vi "pallindrome.vi"() -> ()   [LabVIEW 2018]
panel:
  out "Numeric":dbl
  out "PALLINDROME OR NOT":string
  out "Boolean":bool
  in  "String":string
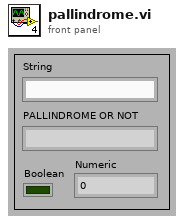
[diagram p1: front panel]
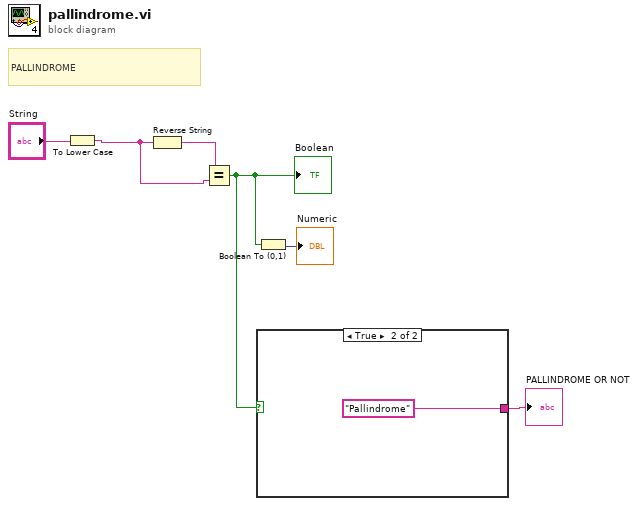
[diagram p0: block diagram]
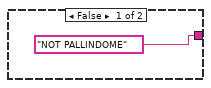
[diagram p2: hidden frame]
diagram:
  # "PALLINDROME"
  n1 = To Lower Case(string="String") -> (all lower case string=w3:string)
  n2 = Reverse String(1:w3) -> (0:w6:string)
  n3 = Equal?(x=w6, y=w3) -> (x = y?=w1:bool)
  "Boolean" <- w1
  n4 = case shown="True" w1 {
    tunnel: ["NOT PALLINDOME" "Pallindrome"] -> w5
    frame False {
    }
    frame True {
    }
  }
  "PALLINDROME OR NOT" <- w5
  n5 = Boolean To (0,1)(Boolean=w1) -> (0, 1=→"Numeric":i16)
